vi "Measurement Logic.vi"(8 "error in":errorcluster, 9 "measurement configuration":T2={"Input Terminal Name"="Lorem ipsum dolor sit", "Counter Interface"="", "Active Edge"=10171, "Pulses"=0, "Timeout (s)"=0} {"Active Edge" items=["Rising"=10280, "Falling"=10171]}, 10 "measure call context in":refnum<class "Measure Call Context.lvclass">) -> (0 "error out":errorcluster, 1 "Measurements Resuts":T1, 2 "measure call context out":refnum<class "Measure Call Context.lvclass">)   [LabVIEW 2025, in "Count Edges.lvclass"]
doc: "Contains the core logic for executing the measurement."
uses:
  Count Edges.lvclass
  <vilib>/Plug-In SDKs/Measurements/Measure Call Context/Measure Call Context.lvclass
  Measurement Configuration.ctl
  Measurement Results.ctl
  <vilib>/DAQmx/read.llb/DAQmx Read (Counter U32 1Chan 1Samp).vi
  <vilib>/DAQmx/create/channels.llb/DAQmx Create Channel (CI-Count Edges).vi
  <vilib>/DAQmx/miscellaneous.llb/DAQmx Fill In Error Info.vi
  <extravilib>/ChannelInstances/Event Messenger-bool/Instantiate.vi
  Count Edges.lvclass/Count Edges.ctl
  <resource>/objmgr/daqmx.rc
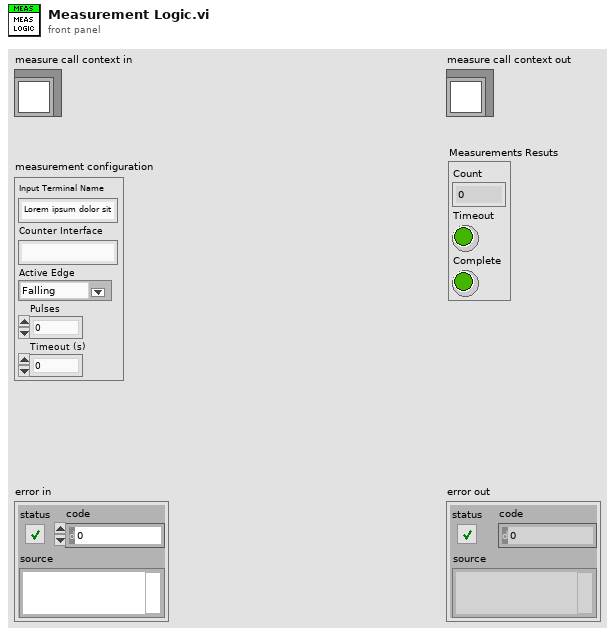
[diagram p1: front panel]
types:
  T1 = typedef "Count Edges.lvclass/Measurement Results.ctl" = cluster{"Count":u32, "Timeout":bool, "Complete":bool}
  T2 = typedef "Count Edges.lvclass/Measurement Configuration.ctl" = cluster{"Input Terminal Name":string, "Counter Interface":string, "Active Edge":i32, "Pulses":u32, "Timeout (s)":u32}
  T3 = typedef "Event Messenger-bool.lvlib/))Channel.ctl" = refnum<queue>
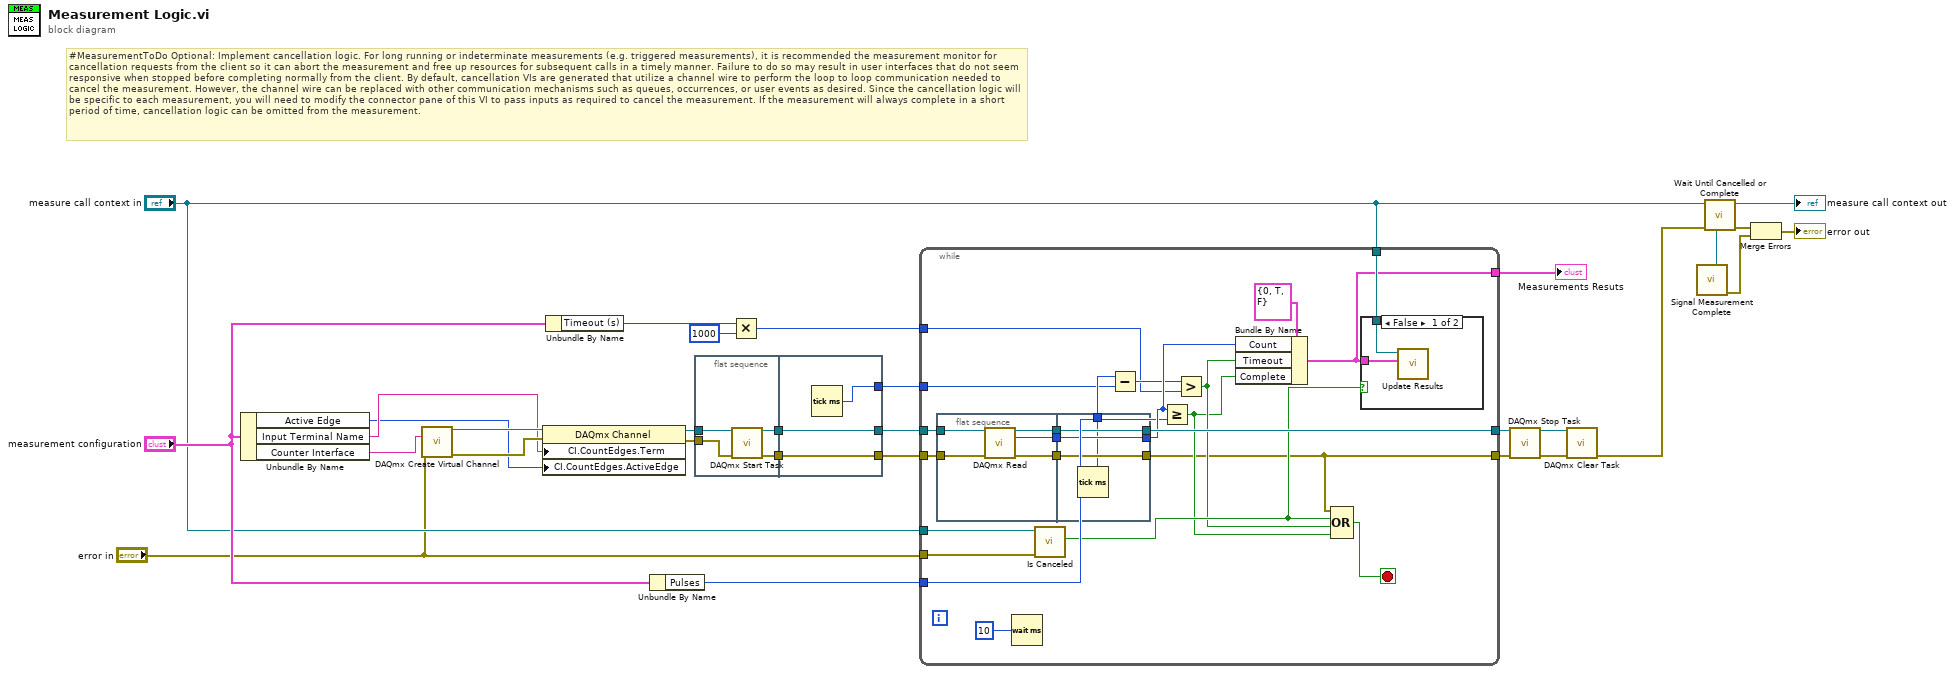
[diagram p0: block diagram]
diagram:
  # "#MeasurementToDo Optional: Implement cancellation logic. For long running or indeterminate measurements (e.g. triggered measurements), it is recommended the measurement monitor for cancellation requests from the client so it can abort the measurement and free up resources for subsequent calls in a timely manner. Failure to do so may result in user interfaces that do not seem responsive when stopped before completing normally from the client. By default, cancellation VIs are generated that utilize a channel wire to perform the loop to loop communication needed to cancel the measurement. However, the channel wire can be replaced with other communication mechanisms such as queues, occurrences, or user events as desired. Since the cancellation logic will be specific to each measurement, you will need to modify the connector pane of this VI to pass inputs as required to cancel the measurement. If the measurement will always complete in a short period of time, cancellation logic can be omitted from the measurement."
  n1 = Unbundle By Name("measurement configuration") -> ("Active Edge"=w15:i32, "Input Terminal Name"=w16:string, "Counter Interface"=w17:string)
  n2 = call-poly <vilib>:"DAQmx Create Virtual Channel.vi"("counter"=w17, "error in"="error in") -> ("task out"=w23:refnum<k21>, "error out"=w22:errorcluster)  [unwired: 12 in]
  n3 = property class="DAQmx Channel"(reference=w23, error in=w22, "CI.CountEdges.Term"=w16, "CI.CountEdges.ActiveEdge"=w15) -> (reference out=w4:refnum<k21>, error out=w25:errorcluster)
  n4 = Unbundle By Name("measurement configuration") -> ("Timeout (s)"=w10:u32)
  n5 = Unbundle By Name("measurement configuration") -> ("Pulses"=w13:u32)
  n6 = flat-sequence {
    tunnel: w25 -> [w34]
    tunnel: [w33] -> w8
    tunnel: [w32] -> w7
    tunnel: w4 -> [w31]
    tunnel: [w37] -> w24
    tunnel: w8 -> [w36]
    tunnel: w7 -> [w37]
    tunnel: [w36] -> w6
    tunnel: [w35] -> w5
    frame #0 {
      n7 = call <vilib>:"DAQmx Start Task.vi"("task/channels in"=w31, "error in"=w34) -> ("task out"=w33:refnum<k21>, "error out"=w32:errorcluster)  [unwired: 12 in]
    }
    frame #1 {
      n8 = Tick Count (ms)() -> (millisecond timer value=w35:u32)
    }
  }
  n9 = Multiply(x=w10, y=u32 1000) -> (x*y=w9:u32)
  n10 = while {
    tunnel: w24 -> [w60]
    tunnel: [w38] -> w20
    tunnel: [w59] -> w21
    tunnel: "error in" -> [w57]
    tunnel: "measure call context in" -> [w56]
    tunnel: w13 -> [w54]
    tunnel: w5 -> [w49]
    tunnel: w9 -> [w47]
    tunnel: w6 -> [w46]
    tunnel: "measure call context in" -> [w44]
    tunnel: [w43] -> w3
    stop <- w39 stop-if-true
    n11 = flat-sequence {
      tunnel: w60 -> [w67]
      tunnel: [w66] -> w53
      tunnel: [w65] -> w52
      tunnel: [w64] -> w51
      tunnel: w46 -> [w63]
      tunnel: [w69] -> w55
      tunnel: [w70] -> w38
      tunnel: [w71] -> w59
      tunnel: w53 -> [w71]
      tunnel: w52 -> [w70]
      tunnel: w51 -> [w69]
      tunnel: [w68] -> w50
      frame #0 {
        n12 = call-poly <vilib>:"DAQmx Read.vi"("task/channels in"=w63, "error in"=w67) -> ("task out"=w66:refnum<k21>, "data"=w64:u32, "error out"=w65:errorcluster)  [unwired: 11 in]
      }
      frame #1 {
        n13 = Tick Count (ms)() -> (millisecond timer value=w68:u32)
      }
    }
    n14 = Wait (ms)(milliseconds to wait=u32 10 ("Loop Time (ms)")) -> ()  [unwired: 1 out]
    n15 = call <vilib>:"Is Canceled.vi"("error in"=w57, "measure call context in"=w56) -> ("is canceled?"=w42:bool)  [unwired: 7 in, 2 out]
    n16 = Subtract(x=w50, y=w49) -> (x-y=w48:u32)
    n17 = Greater Or Equal?(x=w55, y=w54) -> (x >= y?=w40:bool)
    n18 = Greater?(x=w48, y=w47) -> (0:w41:bool)
    n19 = Bundle By Name(cluster=T1 {"Count"=0, "Timeout"=TRUE, "Complete"=FALSE} ("measurement results"), "Count"=w55, "Timeout"=w41, "Complete"=w40) -> (w43:T1)
    n20 = Compound Arithmetic op=OR(w38, w42, w41, w40) -> (w39:bool)
    n21 = case shown="False" w42 {
      tunnel: w43 -> [w62 _]
      tunnel: w44 -> [w61 _]
      frame False {
        n22 = call <vilib>:"Update Results.vi"("measurement results"=w62, "measure call context in"=w61) -> ()  [unwired: 8 in, 2 out]
      }
      frame True {
      }
    }
  }
  "Measurements Resuts" <- w3
  n23 = call <vilib>:"DAQmx Stop Task.vi"("task/channels in"=w21, "error in"=w20) -> ("task out"=w18:refnum<k21>, "error out"=w19:errorcluster)  [unwired: 12 in]
  n24 = call <vilib>:"DAQmx Clear Task.vi"("task in"=w18, "error in"=w19) -> ("error out"=w14:errorcluster)  [unwired: 13 in]
  n25 = call "Signal Measurement Complete.vi"() -> ("error out"=w28:errorcluster, "done channel"=w29:T3)  [unwired: 10 in]
  n26 = call "Wait Until Cancelled or Complete.vi"("done channel"=w29, "error in (no error)"=w14, "measure call context in"="measure call context in") -> ("error out"=w27:errorcluster, "measure call context out"=→"measure call context out":refnum<class "Measure Call Context.lvclass">)  [unwired: 7 in]
  n27 = Merge Errors(w27, w28) -> (→"error out":errorcluster)
